vi "Get All Controls.vi"(8 "error in (no error)":errorcluster, 11 "VI":path) -> (0 "error out":errorcluster, 3 "VIs Controls":T1[](array[typedef]))   [LabVIEW 2019, in "Language Editor.lvlib"]
doc: "- - -\nCopyright (c) 2026, Merecs Engineering GmbH"
uses:
  Language Editor.lvlib
  type defs/Cluster VI controls.ctl
panel:
  # "Connector Pane"
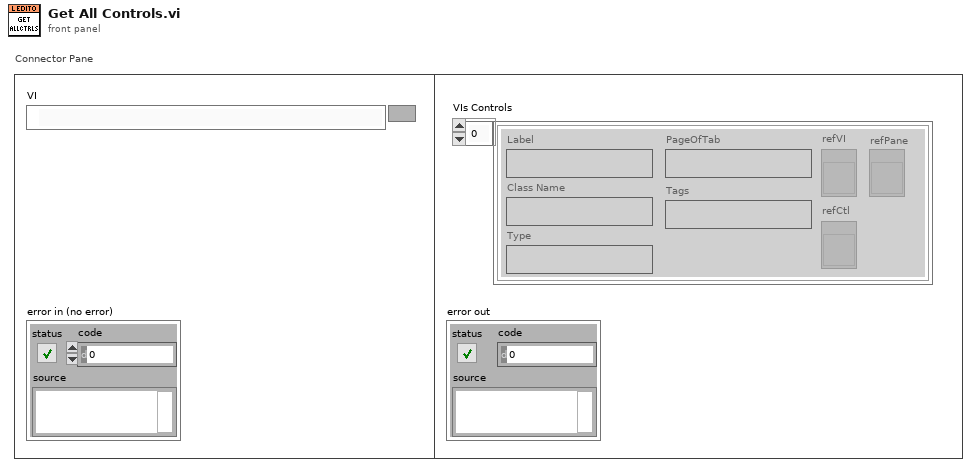
[diagram p1: front panel]
types:
  T1 = typedef "Language Editor.lvlib/Cluster VI controls.ctl" = cluster{"Label":string, "Class Name":string, "Type":string, "Tags":string, "refVI":refnum<vi>, "refCtl":refnum<vi>, "PageOfTab":string, "refPane":refnum<vi>}
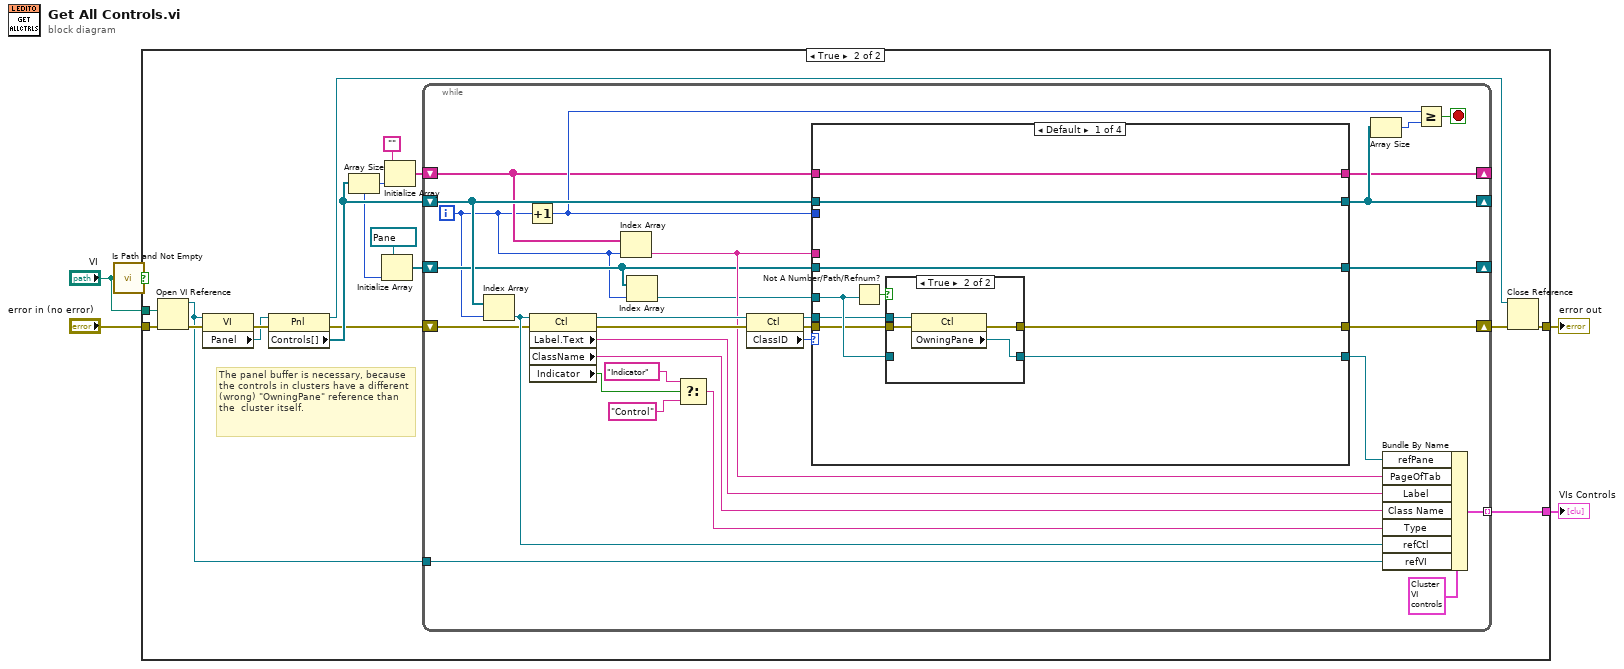
[diagram p0: block diagram]
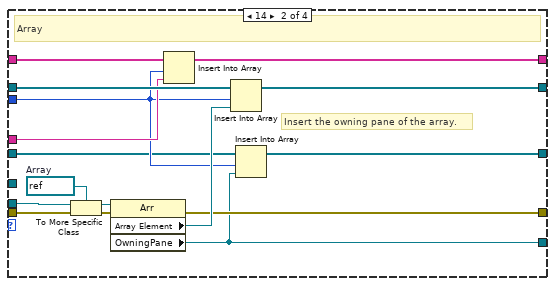
[diagram p4: hidden frame]
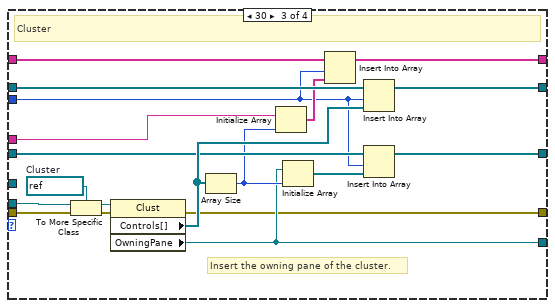
[diagram p5: hidden frame]
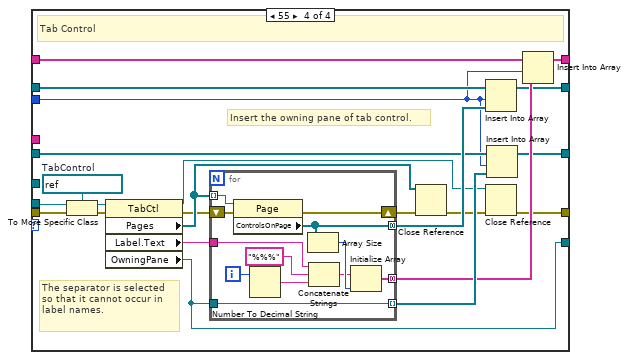
[diagram p6: hidden frame]
diagram:
  n1 = call <vilib>:"Is Path and Not Empty.vi"("path"="VI") -> ("Is Path and Not Empty?"=w2:bool)  [unwired: 4 in]
  n2 = case shown="True" w2 {
    tunnel: "VI" -> [_ w21]
    tunnel: "error in (no error)" -> [w6 w20]
    tunnel: [w6 w17] -> w5
    tunnel: [_ w18] -> w1
    frame False {
    }
    frame True {
      # "The panel buffer is necessary, because the controls in clusters have a different (wrong) \"OwningPane\" reference than the  cluster itself."
      n3 = Open VI Reference(vi path=w21, error in (no error)=w20) -> (vi reference=w7:refnum<vi>, error out=w22:errorcluster)  [unwired: 4 in]
      n4 = property class="VI"(reference=w7, error in=w22) -> (error out=w23:errorcluster, "Panel"=w13:refnum<vi>)  [unwired: 1 out]
      n5 = property class="Pnl"(reference=w13, error in=w23) -> (reference out=w8:refnum<vi>, error out=w9:errorcluster, "Controls[]"=w15:refnum<vi>[])
      n6 = Array Size(array=w15) -> (size(s)=w12:i32)
      n7 = Initialize Array(refnum<vi> refnum ("OwningPane"), w12) -> (w11:refnum<vi>[])
      n8 = Initialize Array("", w12) -> (w14:string[])
      n9 = while {
        shift-right: [w40] -> w19
        shift-left: w9 -> [w36]
        tunnel: [w53] -> w18 mode=indexing
        tunnel: w7 -> [w52]
        shift-right: [w35] -> _
        shift-left: w15 -> [w38]
        shift-right: [w31] -> _
        shift-left: w14 -> [w30]
        shift-right: [w28] -> _
        shift-left: w11 -> [w27]
        i -> [w26]
        stop <- w32 stop-if-true
        n10 = Index Array(array=w38, index=w26) -> (element=w44:refnum<vi>)
        n11 = Increment(x=w26) -> (x+1=w33:i32)
        n12 = property class="Ctl"(reference=w44, error in=w36) -> (reference out=w43:refnum<vi>, error out=w42:errorcluster, "Label.Text"=w47:string, "ClassName"=w46:string, "Indicator"=w51:bool)
        n13 = Index Array(array=w30, index=w26) -> (element=w29:string)
        n14 = Index Array(array=w27, index=w26) -> (element=w25:refnum<vi>)
        n15 = Select(t="Indicator", s=w51, f="Control") -> (s? t:f=w45:string)
        n16 = property class="Ctl"(reference=w43, error in=w42) -> (reference out=w37:refnum<vi>, error out=w39:errorcluster, "ClassID"=w41:u32)
        n17 = case shown="Default" w41 {
          tunnel: [w57 w76 w85 w113] -> w40
          tunnel: w39 -> [w58 w83 w102 w122]
          tunnel: [w61 w77 w97 w118] -> w35
          tunnel: w38 -> [w61 w79 w98 w108]
          tunnel: w37 -> [w59 w84 w103 w123]
          tunnel: w33 -> [_ w71 w87 w106]
          tunnel: [w60 w74 w95 w110] -> w31
          tunnel: w30 -> [w60 w75 w96 w111]
          tunnel: w29 -> [_ w73 w92 _]
          tunnel: [w56 w70 w86 w104] -> w24
          tunnel: w27 -> [w55 w69 w91 w107]
          tunnel: [w55 w72 w90 w105] -> w28
          tunnel: w25 -> [w62 _ _ _]
          frame Default {
            n18 = Not A Number/Path/Refnum?(number/path/refnum=w62) -> (NaN/Path/Refnum?=w54:bool)
            n19 = case shown="True" w54 {
              tunnel: w59 -> [_ w68]
              tunnel: w58 -> [w64 w67]
              tunnel: [w64 w66] -> w57
              tunnel: [w63 w65] -> w56
              tunnel: w62 -> [w63 _]
              frame False {
              }
              frame True {
                n20 = property class="Ctl"(reference=w68, error in=w67) -> (error out=w66:errorcluster, "OwningPane"=w65:refnum<vi>)  [unwired: 1 out]
              }
            }
          }
          frame 14 {
            w82 = refnum<vi> refnum  # Array
            # "Insert the owning pane of the array."
            # "Array"
            n21 = To More Specific Class(target class=w82, reference=w84, error in=w83) -> (specific class reference=w81:refnum<vi>, error out=w80:errorcluster)
            n22 = property class="Arr"(reference=w81, error in=w80) -> (error out=w76:errorcluster, "Array Element"=w78:refnum<vi>, "OwningPane"=w70:refnum<vi>)  [unwired: 1 out]
            n23 = Insert Into Array(array=w75, index=w71, new element=w73) -> (w74:string[])
            n24 = Insert Into Array(array=w79, index=w71, new element=w78) -> (w77:refnum<vi>[])
            n25 = Insert Into Array(array=w69, index=w71, new element=w70) -> (w72:refnum<vi>[])
          }
          frame 30 {
            w101 = refnum<vi> refnum  # Cluster
            # "Insert the owning pane of the cluster."
            # "Cluster"
            n26 = To More Specific Class(target class=w101, reference=w103, error in=w102) -> (specific class reference=w100:refnum<vi>, error out=w99:errorcluster)
            n27 = property class="Clust"(reference=w100, error in=w99) -> (error out=w85:errorcluster, "Controls[]"=w94:refnum<vi>[], "OwningPane"=w86:refnum<vi>)  [unwired: 1 out]
            n28 = Array Size(array=w94) -> (size(s)=w89:i32)
            n29 = Initialize Array(w92, w89) -> (w93:string[])
            n30 = Initialize Array(w86, w89) -> (w88:refnum<vi>[])
            n31 = Insert Into Array(array=w96, index=w87, new element=w93) -> (w95:string[])
            n32 = Insert Into Array(array=w98, index=w87, new element=w94) -> (w97:refnum<vi>[])
            n33 = Insert Into Array(array=w91, index=w87, new element=w88) -> (w90:refnum<vi>[])
          }
          frame 55 {
            w121 = refnum<vi> refnum  # TabControl
            # "Insert the owning pane of tab control."
            # "The separator is selected so that it cannot occur in label names."
            # "Tab Control"
            n34 = To More Specific Class(target class=w121, reference=w123, error in=w122) -> (specific class reference=w120:refnum<vi>, error out=w119:errorcluster)
            n35 = property class="TabCtl"(reference=w120, error in=w119) -> (reference out=w112:refnum<vi>, error out=w116:errorcluster, "Pages"=w124:refnum<vi>[], "Label.Text"=w109:string, "OwningPane"=w104:refnum<vi>)
            n36 = for {
              tunnel: w124 -> [w138] mode=indexing
              tunnel: [w130] -> w117 mode=concatenating
              shift-right: [w136] -> w115
              shift-left: w116 -> [w137]
              tunnel: [w129] -> w125 mode=concatenating
              tunnel: w109 -> [w132]
              tunnel: [w127] -> w126 mode=indexing
              tunnel: w104 -> [w127]
              i -> [w134]
              n37 = property class="Page"(reference=w138, error in=w137) -> (error out=w136:errorcluster, "ControlsOnPage"=w130:refnum<vi>[])  [unwired: 1 out]
              n38 = Number To Decimal String(number=w134) -> (decimal integer string=w133:string)  [unwired: 1 in]
              n39 = Array Size(array=w130) -> (size(s)=w131:i32)
              n40 = Concatenate Strings(w132, "%%%" ("string"), w133) -> (w128:string)
              n41 = Initialize Array(w128, w131) -> (w129:string[])
            }
            n42 = Close Reference(reference=w124, error in (no error)=w115) -> (error out=w114:errorcluster)
            n43 = Insert Into Array(array=w108, index=w106, new element=w117) -> (w118:refnum<vi>[])
            n44 = Close Reference(reference=w112, error in (no error)=w114) -> (error out=w113:errorcluster)
            n45 = Insert Into Array(array=w107, index=w106, new element=w126) -> (w105:refnum<vi>[])
            n46 = Insert Into Array(array=w111, index=w106, new element=w125) -> (w110:string[])
          }
        }
        n47 = Array Size(array=w35) -> (size(s)=w34:i32)
        n48 = Bundle By Name(cluster=T1 {"Label"="", "Class Name"="", "Type"="", "Tags"="", "refVI"=refnum, "refCtl"=refnum, "PageOfTab"="", "refPane"=refnum} ("VI Control"), "refPane"=w24, "PageOfTab"=w29, "Label"=w47, "Class Name"=w46, "Type"=w45, "refCtl"=w44, "refVI"=w52) -> (w53:T1)
        n49 = Greater Or Equal?(x=w33, y=w34) -> (x >= y?=w32:bool)
      }
      n50 = Close Reference(reference=w8, error in (no error)=w19) -> (error out=w17:errorcluster)
    }
  }
  "error out" <- w5
  "VIs Controls" <- w1
